vi "test tools call mcp names.vi"(8 "error in (no error)":errorcluster) -> (0 "error out":errorcluster, 3 "body":string)   [LabVIEW 2020, in "MCP Server tests.lvlib"]
doc: "tools/call with the MCP names of a tool's inputs reaches the controls behind them, although their labels contain upper case letters, spaces, brackets and special characters, and the output comes back under its MCP name. fake_tool_special_labels multiplies Length (mm) with Factor #1 & 50% into Result (mm): length__mm_ 2.5 and factor__1___50_ 4 give result__mm_ 10. A wrong value proves that a label was not reached."
uses:
  MCP Server tests.lvlib
  14b6674f-7439-499c-a4ad-86df86b5fbb6.vi
  <vilib>/JDP Science/JSONtext/Next JSON Value.vi
  <vilib>/JDP Science/JSONtext/String Subset.vi
  <vilib>/JDP Science/JSONtext/Parsing/Advance past next JSON Value (inlined COPY).vi
  <vilib>/JDP Science/JSONtext/Parsing/Advance past whitespace.vi
  <vilib>/JDP Science/JSONtext/Parsing/Advance past String.vi
  <vilib>/JDP Science/JSONtext/Parsing/Advance past Number.vi
  <vilib>/JDP Science/JSONtext/Parsing/Advance past Line Ending.vi
  <vilib>/JDP Science/JSONtext/Parsing/Parse Full Path or Item Name.vi
  <vilib>/JDP Science/JSONtext/Parsing/Advance past Array.vi
  <vilib>/JDP Science/JSONtext/Parsing/Advance past Object.vi
  <vilib>/JDP Science/JSONtext/support/Error Cluster From Code.vi
  <vilib>/JDP Science/JSONtext/Offset/Find Item Locations by Path.vi
  <vilib>/JDP Science/JSONtext/JSON text to Variant.vi
  <vilib>/JDP Science/JSONtext/LVClass Serializer/JSONtext LVClass Serializer.lvclass
  <vilib>/addons/_JKI Toolkits/Caraya/classes/Test/Test.lvclass
  <vilib>/JDP Science/JSONtext/JSONtext.lvlib
  <vilib>/addons/_JKI Toolkits/Caraya/classes/Assert/Assert.lvclass
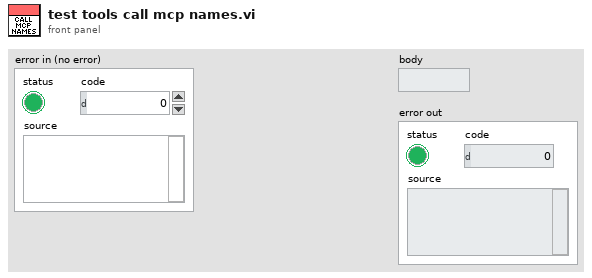
[diagram p1: front panel]
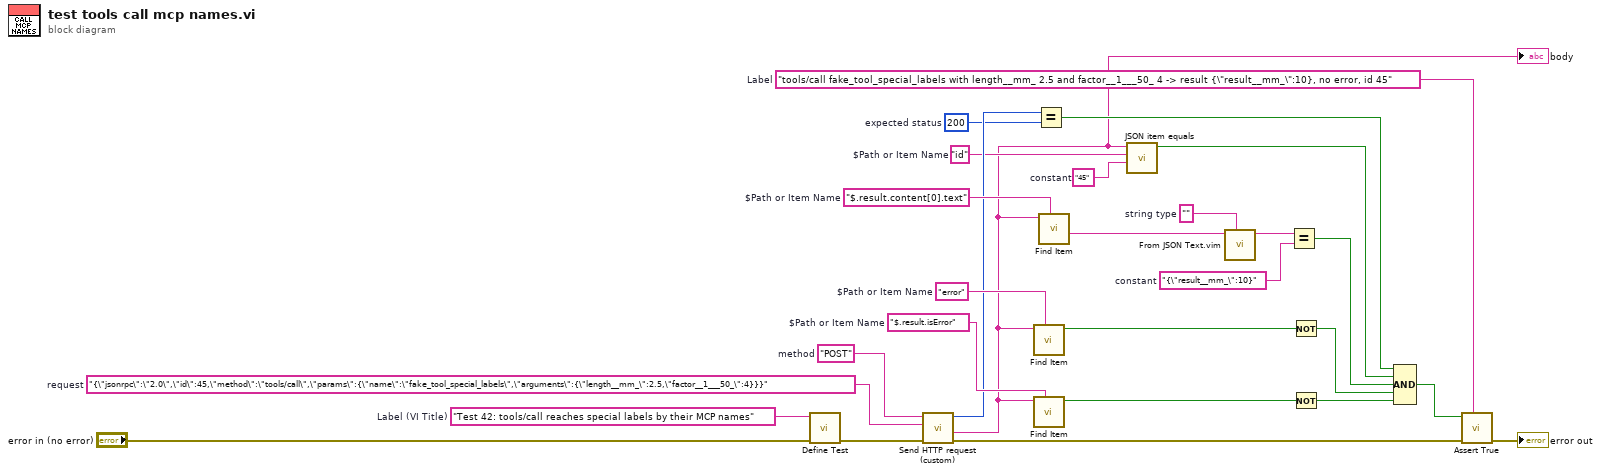
[diagram p0: block diagram]
diagram:
  w3 = "tools/call fake_tool_special_labels with length__mm_ 2.5 and factor__1___50_ 4 -> result {\"result__mm_\":10}, no error, id 45"  # Label
  w11 = "{\"result__mm_\":10}"  # constant
  w15 = ""  # string type
  w17 = "45"  # constant
  w21 = "$.result.isError"  # $Path or Item Name
  w22 = "error"  # $Path or Item Name
  w23 = "$.result.content[0].text"  # $Path or Item Name
  w18 = "id"  # $Path or Item Name
  w19 = 200  # expected status
  w25 = "{\"jsonrpc\":\"2.0\",\"id\":45,\"method\":\"tools/call\",\"params\":{\"name\":\"fake_tool_special_labels\",\"arguments\":{\"length__mm_\":2.5,\"factor__1___50_\":4}}}"  # request
  w26 = "POST"  # method
  w28 = "Test 42: tools/call reaches special labels by their MCP names"  # Label (VI Title)
  n1 = call <vilib>:"Define Test.vi"("error in (no error)"="error in (no error)", "Label (VI Title)"=w28) -> ("error out"=w24:errorcluster)  [unwired: 8 in, 1 out]
  n2 = call "Send HTTP request (custom).vi"("error in (no error)"=w24, "request"=w25, "method"=w26) -> ("error out"=w4:errorcluster, "response"=w2:string, "status code"=w20:i32)  [unwired: 5 in, 1 out]
  "body" <- w2
  n3 = call <vilib>:"Find Item.vi"("$Path or Item Name"=w22, "JSON"=w2) -> ("Found"=w14:bool)  [unwired: 6 in, 3 out]
  n4 = call <vilib>:"Find Item.vi"("$Path or Item Name"=w21, "JSON"=w2) -> ("Found"=w13:bool)  [unwired: 6 in, 3 out]
  n5 = Equal?(x=w20, y=w19) -> (x = y?=w10:bool)
  n6 = call <vilib>:"Find Item.vi"("$Path or Item Name"=w23, "JSON"=w2) -> ("<JSON>"=w16:string)  [unwired: 6 in, 3 out]
  n7 = call "JSON item equals.vi"("expected"=w17, "path"=w18, "JSON"=w2) -> ("equal?"=w9:bool)  [unwired: 6 in, 2 out]
  n8 = call "From JSON Text.vim"("Data Type and Default Value"=w15, "JSON"=w16) -> ("Data out"=w12:string)  [unwired: 8 in, 1 out]
  n9 = Equal?(x=w12, y=w11) -> (x = y?=w8:bool)
  n10 = Not(x=w14) -> (.not. x?=w7:bool)
  n11 = Not(x=w13) -> (.not. x?=w6:bool)
  n12 = Compound Arithmetic op=AND(w10, w9, w8, w7, w6) -> (w5:bool)
  n13 = call <vilib>:"Assert True.vi"("Label"=w3, "error in (no error)"=w4, "True?"=w5) -> ("error out"=→"error out":errorcluster)  [unwired: 7 in, 1 out]
